vi "RemoteVI Caraya Runner.vi"(0 "Report Path":path) -> (4 "Report Path used":path, 15 "error out":errorcluster)   [LabVIEW 2020]
doc: "Runs every RemoteVI Caraya unit test (generated by tests/caraya/build.py) with Caraya's Run Tests (Array Path), non-interactive, and writes a JUnit report. Test paths are relative to this VI, so the folder can move. Report Path empty: RemoteVI Caraya Report.xml beside this VI. Caraya answers 7002 in error out when a test failed - read the report for which one."
uses:
  <vilib>/addons/_JKI Toolkits/Caraya/Caraya.lvlib
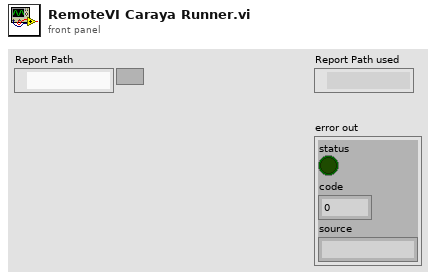
[diagram p1: front panel]
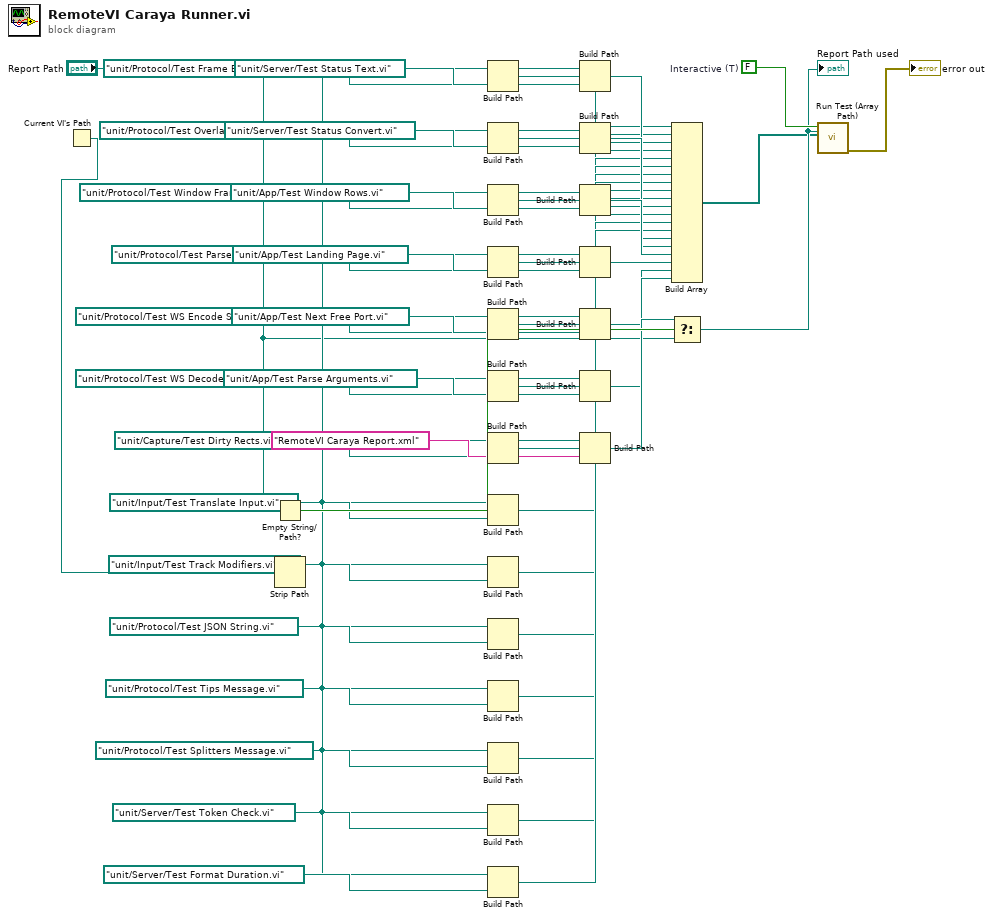
[diagram p0: block diagram]
diagram:
  w49 = FALSE  # Interactive (T)
  n1 = Current VI's Path() -> (path=w2:path)
  n2 = Empty String/Path?(string/path="Report Path") -> (empty?=w47:bool)
  n3 = Strip Path(path=w2) -> (stripped path=w3:path)  [unwired: 1 out]
  n4 = Build Path(base path=w3, name or relative path=path "unit/Protocol/Test Frame Encode.vi") -> (appended path=w5:path)
  n5 = Build Path(base path=w3, name or relative path=path "unit/Protocol/Test Overlay Encode.vi") -> (appended path=w7:path)
  n6 = Build Path(base path=w3, name or relative path=path "unit/Protocol/Test Window Frame Encode.vi") -> (appended path=w9:path)
  n7 = Build Path(base path=w3, name or relative path=path "unit/Protocol/Test Parse Input.vi") -> (appended path=w11:path)
  n8 = Build Path(base path=w3, name or relative path=path "unit/Protocol/Test WS Encode Server Frame.vi") -> (appended path=w13:path)
  n9 = Build Path(base path=w3, name or relative path=path "unit/Protocol/Test WS Decode Client Frame.vi") -> (appended path=w15:path)
  n10 = Build Path(base path=w3, name or relative path=path "unit/Capture/Test Dirty Rects.vi") -> (appended path=w17:path)
  n11 = Build Path(base path=w3, name or relative path=path "unit/Input/Test Translate Input.vi") -> (appended path=w19:path)
  n12 = Build Path(base path=w3, name or relative path=path "unit/Input/Test Track Modifiers.vi") -> (appended path=w21:path)
  n13 = Build Path(base path=w3, name or relative path=path "unit/Protocol/Test JSON String.vi") -> (appended path=w23:path)
  n14 = Build Path(base path=w3, name or relative path=path "unit/Protocol/Test Tips Message.vi") -> (appended path=w25:path)
  n15 = Build Path(base path=w3, name or relative path=path "unit/Protocol/Test Splitters Message.vi") -> (appended path=w27:path)
  n16 = Build Path(base path=w3, name or relative path=path "unit/Server/Test Token Check.vi") -> (appended path=w29:path)
  n17 = Build Path(base path=w3, name or relative path=path "unit/Server/Test Format Duration.vi") -> (appended path=w31:path)
  n18 = Build Path(base path=w3, name or relative path=path "unit/Server/Test Status Text.vi") -> (appended path=w33:path)
  n19 = Build Path(base path=w3, name or relative path=path "unit/Server/Test Status Convert.vi") -> (appended path=w35:path)
  n20 = Build Path(base path=w3, name or relative path=path "unit/App/Test Window Rows.vi") -> (appended path=w37:path)
  n21 = Build Path(base path=w3, name or relative path=path "unit/App/Test Landing Page.vi") -> (appended path=w39:path)
  n22 = Build Path(base path=w3, name or relative path=path "unit/App/Test Next Free Port.vi") -> (appended path=w41:path)
  n23 = Build Path(base path=w3, name or relative path=path "unit/App/Test Parse Arguments.vi") -> (appended path=w43:path)
  n24 = Build Path(base path=w3, name or relative path="RemoteVI Caraya Report.xml") -> (appended path=w46:path)
  n25 = Build Array(w5, w7, w9, w11, w13, w15, w17, w19, w21, w23, w25, w27, w29, w31, w33, w35, w37, w39, w41, w43) -> (w44:path[])
  n26 = Select(t=w46, s=w47, f="Report Path") -> (s? t:f=w48:path)
  "Report Path used" <- w48
  n27 = call <vilib>:"Run Test (Array Path).vi"("Report Path"=w48, "Paths"=w44, "Interactive (T)"=w49) -> ("error out"=→"error out":errorcluster)  [unwired: 7 in, 1 out]
